vi "Insert into Subpanel.vi"(8 "error in (no error)":errorcluster, 10 "SubPanel":refnum<vi>, 11 "Express VI Type in":refnum<class "Express VI Type.lvclass">) -> (0 "error out":errorcluster, 3 "Express VI Type out":refnum<class "Express VI Type.lvclass">)   [LabVIEW 2020, in "Peek Window.lvlib" / "Express VI Type.lvclass"]
uses:
  Express VI Type.lvclass
  Express VI Type.lvclass/Express VI Type.ctl
  Standard VI Type/Standard VI Type.lvclass/Standard VI Type.ctl
  Standard VI Type/Read VI Refnum.vi
  Implementation VI Type/Implementation VI Type.lvclass
  D:/Code/VI-Peek/source/Peek Window/VI Types/Standard VI Type/Standard VI Type.lvclass
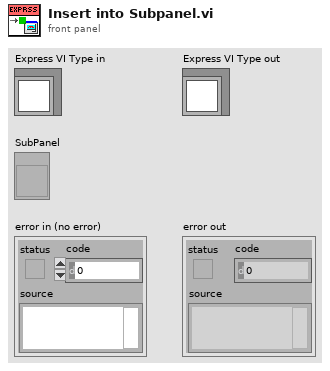
[diagram p1: front panel]
types:
  T1 = enum8{"Enabled", "Disabled", "Disabled and Grayed Out"}
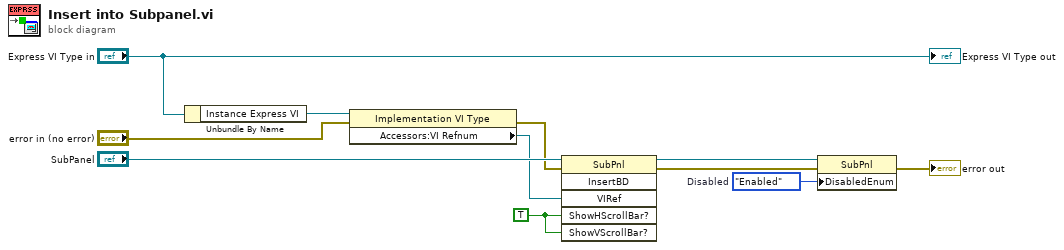
[diagram p0: block diagram]
diagram:
  w4 = T1."Enabled"  # Disabled
  w11 = TRUE ("ShowHScrollBar")
  n1 = Unbundle By Name("Express VI Type in") -> ("Instance Express VI"=w8:refnum<class "Implementation VI Type.lvclass">)
  n2 = property class="Implementation VI Type"(reference=w8, error in="error in (no error)") -> (error out=w5:errorcluster, "Accessors:VI Refnum"=w7:refnum<vi>)  [unwired: 1 out]
  n3 = invoke on="Invoke Node" class="SubPnl" method="InsertBD"(reference="SubPanel", error in=w5, "VIRef"=w7, "ShowHScrollBar?"=w11, "ShowVScrollBar?"=w11) -> (reference out=w1:refnum<vi>, error out=w3:errorcluster)  [unwired: 1 in, 4 out]
  n4 = property class="SubPnl"(reference=w1, error in=w3, "DisabledEnum"=w4) -> (error out=→"error out":errorcluster)  [unwired: 1 out]
  "Express VI Type out" <- "Express VI Type in"
